vi "VIH Project Tree - Item Type to Boolean Flags.vi"(11 "Item Type":T1) -> (0 "VI with Conpane":bool, 1 "Dynamic":bool, 2 "Palette menu":bool, 3 "Can be built":bool, 4 "Built In Function":bool, 5 "Can be opened":bool, 7 "Can be Removed":bool)   [LabVIEW 2014]
doc: "::: VI Helpeks :::\nCopyright (c) 2000-2026 Konstantin Shifershteyn. All rights reserved."
uses:
  VIH Project Tree Typedef - Tree Item Type.ctl
panel:
  # "VI Helpeks\nCopyright (c) 2012-2026 Konstantin Shifershteyn"
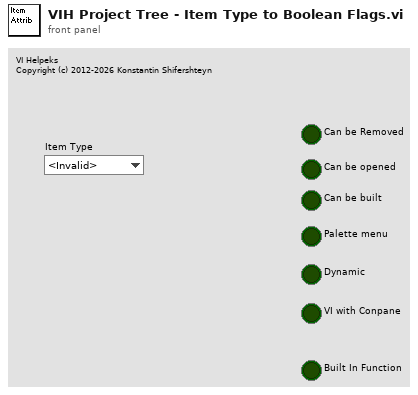
[diagram p1: front panel]
types:
  T1 = typedef "VIH Project Tree Typedef - Tree Item Type.ctl" = enum32{"<Invalid>", "Project", "Proj Files", "Proj Rules", "File Group", "Rule Group", "Any File", "LV Func", ".mnu", ".mnu (dyn)", ".vi", ".vi (dyn)", ".vit", ".vit (dyn)", ".ctl", ".ctl (dyn)", ".ctt", ".ctt (dyn)", "polyVI", "polyVI (dyn)", "expVI", "expVI (dyn)", "HTML", "PolyVI Inst"}
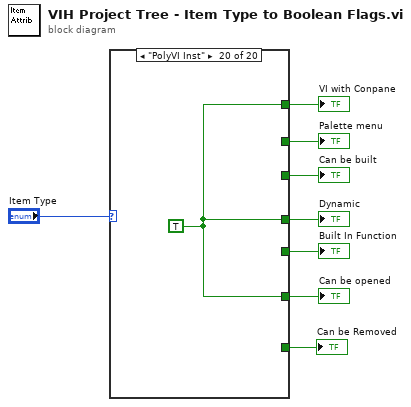
[diagram p0: block diagram]
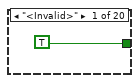
[diagram p2: hidden frame]
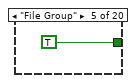
[diagram p6: hidden frame]
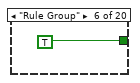
[diagram p7: hidden frame]
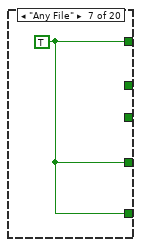
[diagram p8: hidden frame]
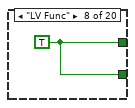
[diagram p9: hidden frame]
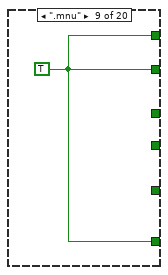
[diagram p10: hidden frame]
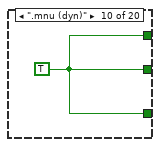
[diagram p11: hidden frame]
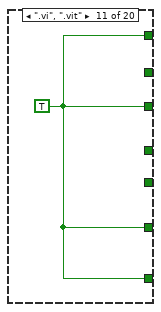
[diagram p12: hidden frame]
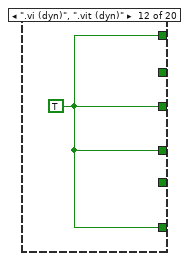
[diagram p13: hidden frame]
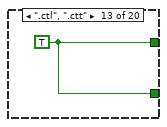
[diagram p14: hidden frame]
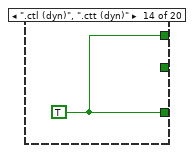
[diagram p15: hidden frame]
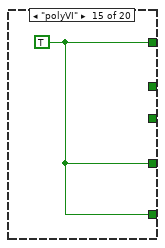
[diagram p16: hidden frame]
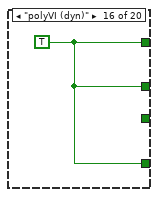
[diagram p17: hidden frame]
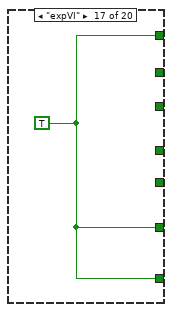
[diagram p18: hidden frame]
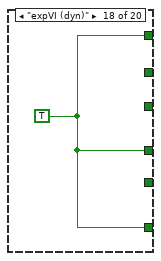
[diagram p19: hidden frame]
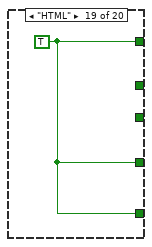
[diagram p20: hidden frame]
diagram:
  n1 = case shown="\"PolyVI Inst\"" "Item Type" {
    tunnel: [_ _ _ _ _ _ _ _ w14 w15 _ _ _ _ _ _ _ _ _ _] -> w7
    tunnel: [_ _ _ _ _ _ w12 _ w14 w15 w16 w17 _ _ w20 w21 _ _ w24 _] -> w8
    tunnel: [_ _ _ _ _ _ _ w13 _ w15 _ w17 _ w19 _ w21 _ w23 _ w25] -> w5
    tunnel: [_ _ _ _ _ _ _ w13 _ _ _ _ _ _ _ _ _ _ _ _] -> w4
    tunnel: [_ _ _ _ _ _ _ _ _ _ w16 w17 _ _ _ _ w22 w23 _ w25] -> w3
    tunnel: [_ _ _ _ _ _ w12 _ _ _ w16 w17 w18 w19 w20 w21 w22 w23 w24 w25] -> w2
    tunnel: [TRUE _ _ _ TRUE TRUE w12 _ w14 _ w16 _ w18 _ w20 _ w22 _ w24 _] -> w1
    frame "<Invalid>" {
    }
    frame "Project" {
    }
    frame "Proj Files" {
    }
    frame "Proj Rules" {
    }
    frame "File Group" {
    }
    frame "Rule Group" {
    }
    frame "Any File" {
      w12 = TRUE
    }
    frame "LV Func" {
      w13 = TRUE
    }
    frame ".mnu" {
      w14 = TRUE
    }
    frame ".mnu (dyn)" {
      w15 = TRUE
    }
    frame ".vi", ".vit" {
      w16 = TRUE
    }
    frame ".vi (dyn)", ".vit (dyn)" {
      w17 = TRUE
    }
    frame ".ctl", ".ctt" {
      w18 = TRUE
    }
    frame ".ctl (dyn)", ".ctt (dyn)" {
      w19 = TRUE
    }
    frame "polyVI" {
      w20 = TRUE
    }
    frame "polyVI (dyn)" {
      w21 = TRUE
    }
    frame "expVI" {
      w22 = TRUE
    }
    frame "expVI (dyn)" {
      w23 = TRUE
    }
    frame "HTML" {
      w24 = TRUE
    }
    frame "PolyVI Inst" {
      w25 = TRUE
    }
  }
  "Palette menu" <- w7
  "Can be built" <- w8
  "Dynamic" <- w5
  "Built In Function" <- w4
  "Can be opened" <- w2
  "VI with Conpane" <- w3
  "Can be Removed" <- w1
